vi "_Buffer_To_ElementAtIndex.vi"(10 "index":i32=-1 caption="index (-1: last)", 11 "Buffer":refnum<class "VariantBuffer.lvclass">) -> (1 "found":bool, 3 "element":variant)   [LabVIEW 2013, in "CircularBuffer.lvlib" / "VariantBuffer.lvclass"]
uses:
  VariantBuffer.lvclass
  VariantBuffer.lvclass/VariantBuffer.ctl
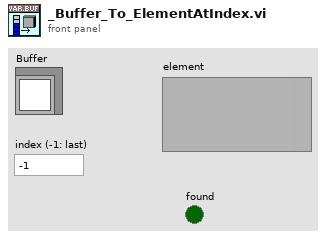
[diagram p1: front panel]
types:
  T1 = typedef "CircularBuffer.lvlib/VariantBuffer.lvclass/buffer-type -- enum.ctl" = enum16{"Queue", "Stack"}
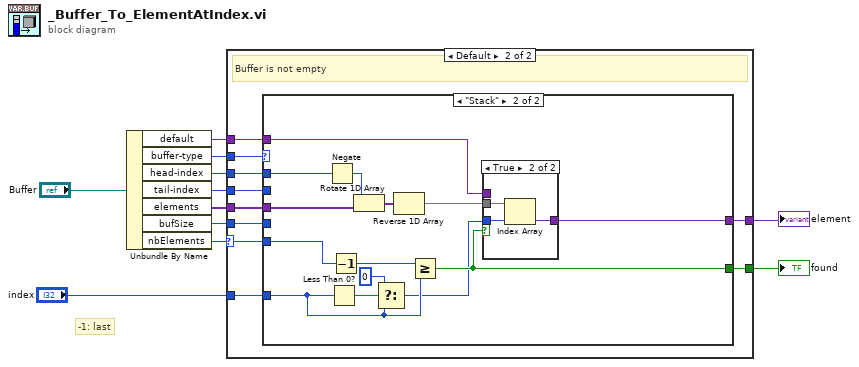
[diagram p0: block diagram]
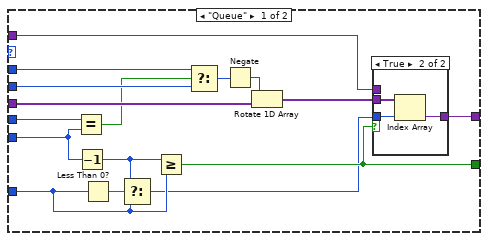
[diagram p3: hidden frame]
diagram:
  # "-1: last"
  n1 = Unbundle By Name("Buffer") -> ("default"=w1:variant, "buffer-type"=w3:T1, "head-index"=w6:i32, "tail-index"=w10:i32, "elements"=w9:variant[], "bufSize"=w11:i32, "nbElements"=w2:i32)
  n2 = case shown="Default" w2 {
    selector: w2 -> [_ w14]
    tunnel: w11 -> [_ w22]
    tunnel: w10 -> [_ w17]
    tunnel: w9 -> [_ w15]
    tunnel: [w12 w21] -> w8
    tunnel: "index" -> [_ w19]
    tunnel: [_ w20] -> w7
    tunnel: w1 -> [w12 w18]
    tunnel: w6 -> [_ w16]
    tunnel: w3 -> [_ w13]
    frame 0 {
      # "Buffer is empty"
    }
    frame Default {
      # "Buffer is not empty"
      n3 = case shown="\"Stack\"" w13 {
        tunnel: w22 -> [w38 _]
        tunnel: [w37 w56] -> w21
        tunnel: [w36 w55] -> w20
        tunnel: w19 -> [w35 w50]
        tunnel: w18 -> [w33 w54]
        tunnel: w17 -> [w32 _]
        tunnel: w16 -> [w31 w53]
        tunnel: w15 -> [w30 w51]
        tunnel: w14 -> [w27 w52]
        frame "Queue" {
          n4 = Equal?(x=w38, y=w27) -> (x = y?=w25:bool)
          n5 = Decrement(x=w27) -> (x-1=w29:i32)
          n6 = Less Than 0?(x=w35) -> (x < 0?=w34:bool)
          n7 = Select(t=w29, s=w34, f=w35) -> (s? t:f=w28:i32)
          n8 = Greater Or Equal?(x=w29, y=w35) -> (x >= y?=w36:bool)
          n9 = Select(t=w31, s=w25, f=w32) -> (s? t:f=w24:i32)
          n10 = Negate(x=w24) -> (-x=w23:i32)
          n11 = Rotate 1D Array(1:w30, 2:w23) -> (0:w26:variant[])
          n12 = case shown="True" w36 {
            tunnel: w26 -> [_ w42]
            tunnel: [w39 w41] -> w37
            tunnel: w28 -> [_ w40]
            tunnel: w33 -> [w39 _]
            frame False {
            }
            frame True {
              n13 = Index Array(array=w42, index=w40) -> (element=w41:variant)
            }
          }
        }
        frame "Stack" {
          n14 = Negate(x=w53) -> (-x=w45:i32)
          n15 = Less Than 0?(x=w50) -> (x < 0?=w49:bool)
          n16 = Decrement(x=w52) -> (x-1=w48:i32)
          n17 = Rotate 1D Array(1:w51, 2:w45) -> (0:w44:variant[])
          n18 = Select(t=0, s=w49, f=w50) -> (s? t:f=w47:i32)
          n19 = Reverse 1D Array(array=w44) -> (reversed array=w46:variant[])
          n20 = Greater Or Equal?(x=w48, y=w50) -> (x >= y?=w55:bool)
          n21 = case shown="True" w55 {
            tunnel: w46 -> [_ w60]
            tunnel: [w57 w59] -> w56
            tunnel: w47 -> [_ w58]
            tunnel: w54 -> [w57 _]
            frame False {
            }
            frame True {
              n22 = Index Array(array=w60, index=w58) -> (element=w59:variant)
            }
          }
        }
      }
    }
  }
  "element" <- w8
  "found" <- w7
